vi "Update I2C Monitor Table.vi"(5 "Status Ref":refnum<vi>, 6 "Transactions Limit (10k)":i32=10000 format="%.0p", 7 "# TXNS IN TABLE Ref":refnum<vi>, 8 "error in (no error)":errorcluster, 10 "I2C Data in":string[][](array[string]), 11 "I2C Table Ref":refnum<vi>) -> (0 "error out":errorcluster)   [LabVIEW 2025, in "I2C Bus Monitor UI.lvlib"]
uses:
  I2C Bus Monitor UI.lvlib
  Error Global.vi
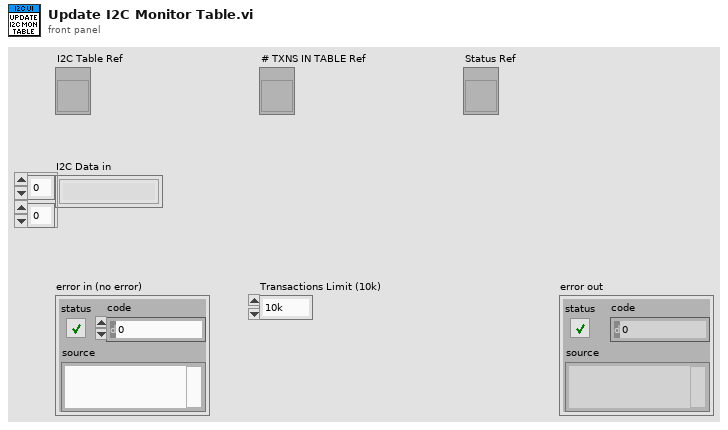
[diagram p1: front panel]
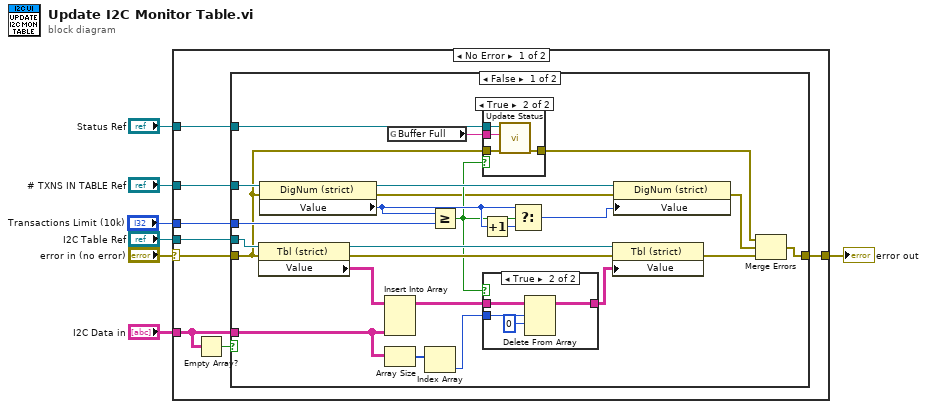
[diagram p0: block diagram]
diagram:
  n1 = case shown="No Error" "error in (no error)" {
    selector: "error in (no error)" -> [w14 w51]
    tunnel: "I2C Table Ref" -> [w15 _]
    tunnel: "I2C Data in" -> [w11 _]
    tunnel: [w13 w51] -> w4
    tunnel: "# TXNS IN TABLE Ref" -> [w10 _]
    tunnel: "Transactions Limit (10k)" -> [w9 _]
    tunnel: "Status Ref" -> [w8 _]
    frame No Error {
      n2 = Empty Array?(array=w11) -> (empty?=w12:bool)
      n3 = case shown="False" w12 {
        tunnel: w11 -> [w18 _]
        tunnel: w15 -> [w39 _]
        tunnel: w14 -> [w25 w50]
        tunnel: [w33 w50] -> w13
        tunnel: w10 -> [w35 _]
        tunnel: w9 -> [w28 _]
        tunnel: w8 -> [w24 _]
        frame False {
          n4 = property on="Property Node" class="Tbl (strict)"(reference=w39, error in=w25) -> (reference out=w38:refnum<vi>, error out=w36:errorcluster, "Value"=w27:string[][])
          n5 = property on="Property Node" class="DigNum (strict)"(reference=w35, error in=w25) -> (reference out=w34:refnum<vi>, error out=w16:errorcluster, "Value"=w30:i32)
          n6 = Insert Into Array(array=w27, new element=w18) -> (w20:string[][])  [unwired: 2 in]
          n7 = Array Size(array=w18) -> (size(s)=w22:i32[])
          n8 = global read "Error Global.vi" "Buffer Full"() -> (w26:string)
          n9 = Index Array(array=w22) -> (element=w17:i32)  [unwired: 1 in]
          n10 = Greater Or Equal?(x=w30, y=w28) -> (x >= y?=w21:bool)
          n11 = Increment(x=w30) -> (x+1=w31:i32)
          n12 = case shown="True" w21 {
            tunnel: w25 -> [w45 w49]
            tunnel: w24 -> [_ w48]
            tunnel: [w45 w47] -> w23
            tunnel: w26 -> [_ w46]
            frame False {
            }
            frame True {
              n13 = call "Update Status.vi"("error in (no error)"=w49, "Value"=w46, "Status Ref"=w48) -> ("error out"=w47:errorcluster)  [unwired: 8 in]
            }
          }
          n14 = case shown="True" w21 {
            tunnel: w20 -> [w40 w44]
            tunnel: [w40 w43] -> w19
            tunnel: w17 -> [_ w42]
            frame False {
            }
            frame True {
              n15 = Delete From Array(array=w44, length=w42, index (row)=0) -> (array with subset deleted=w43:string[][])  [unwired: 1 in, 1 out]
            }
          }
          n16 = Select(t=w30, s=w21, f=w31) -> (s? t:f=w29:i32)
          n17 = property on="Property Node" class="Tbl (strict)"(reference=w38, error in=w36, "Value"=w19) -> (error out=w37:errorcluster)  [unwired: 1 out]
          n18 = property on="Property Node" class="DigNum (strict)"(reference=w34, error in=w16, "Value"=w29) -> (error out=w32:errorcluster)  [unwired: 1 out]
          n19 = Merge Errors(w23, w32, w37) -> (w33:errorcluster)
        }
        frame True {
        }
      }
    }
    frame Error {
    }
  }
  "error out" <- w4
